vi "Get Groups.vi"(8 "error in (no error)":errorcluster, 11 "ParseSVG in":refnum<class "ParseSVG.lvclass">) -> (0 "error out":errorcluster, 3 "ParseSVG out":refnum<class "ParseSVG.lvclass">)   [LabVIEW 2019, in "ParseSVG.lvclass"]
uses:
  ParseSVG.lvclass
  ParseSVG.lvclass/ParseSVG.ctl
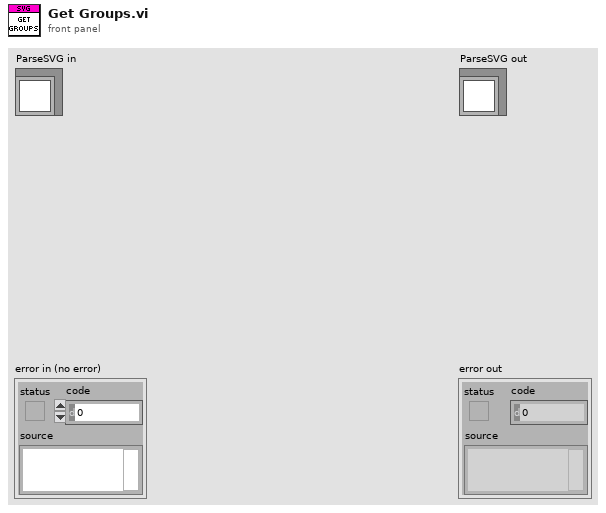
[diagram p1: front panel]
types:
  T1 = cluster{"Start":i32, "id":string, "transforms":string, "End":i32}[]
  T2 = cluster{"offset past match":i32, "RawXML":string}[]
  T3 = cluster{"Start Index":i32, "Data":string, "End Index":i32}
  T4 = cluster{"Start Index":i32, "Data":string, "End Index":i32}[]
  T5 = cluster{"Start Index":i32, "Data":string, "Data":string, "End Index":i32}[]
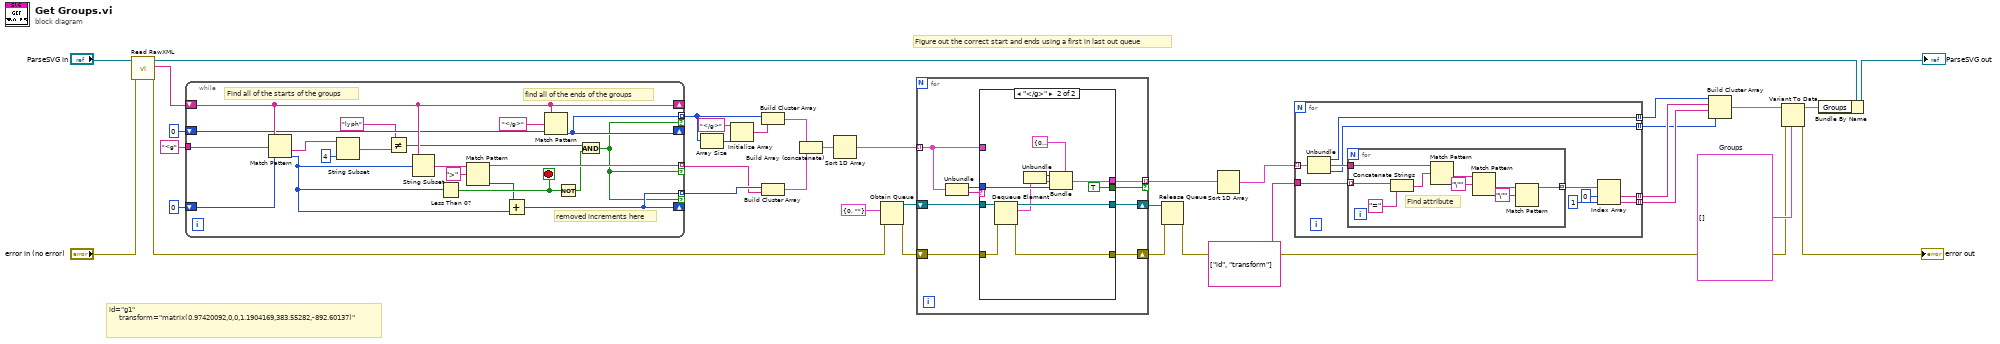
[diagram p0: block diagram]
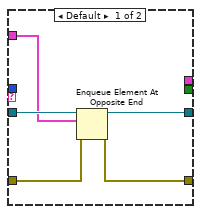
[diagram p2: hidden frame]
diagram:
  w28 = T1 []  # Groups
  # "Figure out the correct start and ends using a first in last out queue"
  # "id=\"g1\"\n     transform=\"matrix(0.97420092,0,0,1.1904169,383.55282,-892.60137)\""
  n1 = call "Read RawXML.vi"("error in (no error)"="error in (no error)", "ParseXML in"="ParseSVG in") -> ("error out"=w12:errorcluster, "RawXML"=w23:string, "ParseXML out"=w26:refnum<class "ParseSVG.lvclass">)  [unwired: 7 in]
  n2 = while {
    shift-right: [w50] -> _
    shift-left: w23 -> [w50]
    shift-right: [w47] -> _
    shift-left: 0 -> [w55]
    tunnel: [w53] -> w16 mode=indexing if=w37
    tunnel: "<g" -> [w44]
    tunnel: [w45] -> w21 mode=indexing if=w37
    tunnel: [w47] -> w17 mode=indexing if=w37
    shift-right: [w45] -> _
    shift-left: 0 ("offset past match") -> [w46]
    stop <- w52 stop-if-true
    # "removed increments here"
    # "Find all of the starts of the groups"
    # "find all of the ends of the groups"
    n3 = Match Pattern(string=w50, regular expression=w44, offset (0)=w55) -> (after substring=w43:string, offset past match=w48:i32)  [unwired: 2 out]
    n4 = String Subset(string=w43, length (rest)=4 ("length (rest)")) -> (substring=w41:string)  [unwired: 1 in]
    n5 = Not Equal?(x="lyph", y=w41) -> (x != y?=w39:bool)
    n6 = String Subset(string=w50, offset (0)=w48) -> (substring=w56:string)  [unwired: 1 in]
    n7 = Less Than 0?(x=w48) -> (x < 0?=w52:bool)
    n8 = Match Pattern(string=w56, regular expression=">") -> (before substring=w53:string, offset past match=w51:i32)  [unwired: 1 in, 2 out]
    n9 = Add(x=w51, y=w48) -> (x+y=w47:i32)
    n10 = Match Pattern(string=w50, regular expression="</g>", offset (0)=w46) -> (offset past match=w45:i32)  [unwired: 3 out]
    n11 = Not(x=w52) -> (.not. x?=w38:bool)
    n12 = And(x=w39, y=w38) -> (x .and. y?=w37:bool)
  }
  n13 = Array Size(array=w21) -> (size(s)=w20:i32)
  n14 = Initialize Array("</g>", w20) -> (w18:string[])
  n15 = Build Cluster Array(w21, w18) -> (w15:cluster{"offset past match":i32, string}[])
  n16 = Build Cluster Array(w17, w16) -> (w14:cluster{i32, "RawXML":string}[])
  n17 = Build Array (concatenate)(w15, w14) -> (w13:T2)
  n18 = Sort 1D Array(array=w13) -> (sorted array=w10:T2)
  n19 = Obtain Queue(element data type=cluster{"Index":i32, "Data":string} {"Index"=0, "Data"=""}, error in (no error)=w12) -> (queue out=w8:refnum<queue>, error out=w11:errorcluster)  [unwired: 3 in, 1 out]
  n20 = for {
    shift-right: [w62] -> w2
    shift-left: w11 -> [w63]
    tunnel: w10 -> [w64] mode=indexing
    shift-right: [w60] -> w3
    shift-left: w8 -> [w61]
    tunnel: [w58] -> w7 mode=indexing if=w57
    n21 = Unbundle(w64) -> ("offset past match"=w59:i32, "RawXML"=w65:string)
    n22 = case shown="\"</g>\"" w65 {
      tunnel: w64 -> [w66 _]
      tunnel: w63 -> [w70 w78]
      tunnel: [w69 w79] -> w62
      tunnel: w61 -> [w68 w81]
      tunnel: [w67 w80] -> w60
      tunnel: w59 -> [_ w77]
      tunnel: [_ w73] -> w58
      tunnel: [_ TRUE] -> w57
      frame Default {
        n23 = Enqueue Element At Opposite End(queue=w68, element=w66, error in (no error)=w70) -> (queue out=w67:refnum<queue>, error out=w69:errorcluster)  [unwired: 1 in, 1 out]
      }
      frame "</g>" {
        n24 = Dequeue Element(queue=w81, error in (no error)=w78) -> (queue out=w80:refnum<queue>, element=w72:cluster{"Index":i32, "Data":string}, error out=w79:errorcluster)  [unwired: 1 in, 1 out]
        n25 = Unbundle(w72) -> ("Index"=w76:i32, "Data"=w75:string)
        n26 = Bundle(cluster=T3 {"Start Index"=0, "Data"="", "End Index"=0}, "Start Index"=w76, "Data"=w75, "End Index"=w77) -> (w73:T3)
      }
    }
  }
  n27 = Release Queue(queue=w3, error in (no error)=w2) -> (error out=w1:errorcluster)  [unwired: 1 in, 2 out]
  n28 = Sort 1D Array(array=w7) -> (sorted array=w6:T4)
  n29 = for {
    tunnel: w6 -> [w91] mode=indexing
    tunnel: string[] ["id", "transform"] -> [w90]
    tunnel: [w86] -> w31 mode=indexing
    tunnel: [w85] -> w30 mode=indexing
    tunnel: [w83] -> w4 mode=indexing
    tunnel: [w82] -> w5 mode=indexing
    n30 = Unbundle(w91) -> ("Start Index"=w83:i32, "Data"=w84:string, "End Index"=w82:i32)
    n31 = for {
      tunnel: w84 -> [w100]
      tunnel: w90 -> [w93] mode=indexing
      tunnel: [w92] -> w89 mode=indexing
      # "Find attribute"
      n32 = Concatenate Strings(w93, "=" ("string")) -> (w95:string)
      n33 = Match Pattern(string=w100, regular expression=w95) -> (after substring=w99:string)  [unwired: 1 in, 3 out]
      n34 = Match Pattern(string=w99, regular expression="\"") -> (after substring=w97:string)  [unwired: 1 in, 3 out]
      n35 = Match Pattern(string=w97, regular expression="\"") -> (before substring=w92:string)  [unwired: 1 in, 3 out]
    }
    n36 = Index Array(array=w89, index #1=0 ("index"), index #2=1 ("index")) -> (element #1=w86:string, element #2=w85:string)
  }
  n37 = Build Cluster Array(w4, w31, w30, w5) -> (w29:T5)
  n38 = Variant To Data(error in=w1, type=w28, Variant=w29) -> (data=w24:T1, error out=→"error out":errorcluster)
  n39 = Bundle By Name(cluster=w26, "Groups"=w24) -> (→"ParseSVG out":refnum<class "ParseSVG.lvclass">)
